vi "Export JUnit.vi"(8 "error in (no error)":errorcluster) -> (0 "error out":errorcluster)   [LabVIEW 2020, in "Test Runner.JUnit.lvclass"]
uses:
  Test Runner.JUnit.lvclass
  classes/Assert/Assert Greater Or Equal_Variant.vi
  classes/Test/Test.lvclass
  classes/Assert/Assert.lvclass
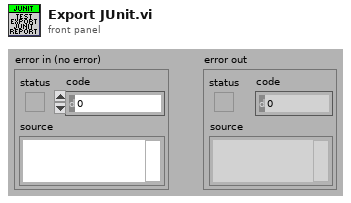
[diagram p1: front panel]
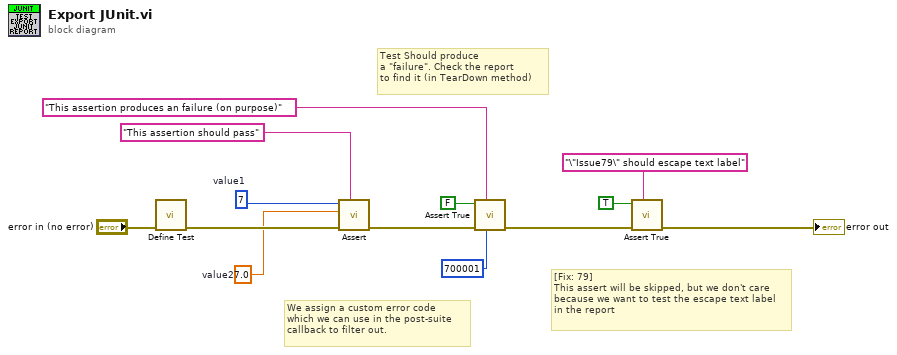
[diagram p0: block diagram]
diagram:
  w2 = 7.0  # value2
  w3 = 7  # value1
  # "We assign a custom error code\nwhich we can use in the post-suite\ncallback to filter out."
  # "[Fix: 79] \nThis assert will be skipped, but we don't care\nbecause we want to test the escape text label\nin the report"
  # "Test Should produce\na \"failure\". Check the report\nto find it (in TearDown method)"
  n1 = call "Define Test.vi"("error in (no error)"="error in (no error)") -> ("error out"=w5:errorcluster)  [unwired: 9 in, 1 out]
  n2 = call-poly "Assert.vi"("Label"="This assertion should pass", "error in (no error)"=w5, "Y"=w2, "X"=w3) -> ("error out"=w4:errorcluster)  [unwired: 6 in, 1 out]
  n3 = call "Assert True.vi"("error code (1)"=700001, "Label"="This assertion produces an failure (on purpose)", "error in (no error)"=w4, "True?"=FALSE) -> ("error out"=w9:errorcluster)  [unwired: 6 in, 1 out]
  n4 = call "Assert True.vi"("Label"="\"Issue79\" should escape text label", "error in (no error)"=w9, "True?"=TRUE) -> ("error out"=→"error out":errorcluster)  [unwired: 7 in, 1 out]
